vi "FIFO.WRITE.vi"(0 "FIFO In":string, 5 "FIFO Name":string, 7 "Data Type":string, 9 "Element":variant, 11 "Input Valid":bool) -> (4 "FIFO Out":string, 6 "Ready for Input":bool)   [LabVIEW 2020]
doc: "Stand-in for an FPGA FIFO Write node with the handshake interface (FIFO In, Element, Input Valid -> Ready for Input, FIFO Out) so that a VI using it can be round-tripped through AIXML. The FIFO's configuration is given as constants on the diagram: FIFO Name (the FIFO item in the LabVIEW project, e.g. TS-Filter.Command) and Data Type (the element type, e.g. orderbook.command.ctl); Element is a Variant so one VI serves every element type (wire the element through To Variant). On My Computer it only passes FIFO In to FIFO Out and reports Ready for Input = TRUE. In the FPGA VI, replace each call with the real FIFO Method Node for FIFO Name and delete the constants."
panel:
  out "Data Type (cfg)":string
  out "FIFO Name (cfg)":string
  out "Input Valid (last)":bool
  out "Element (last)":variant
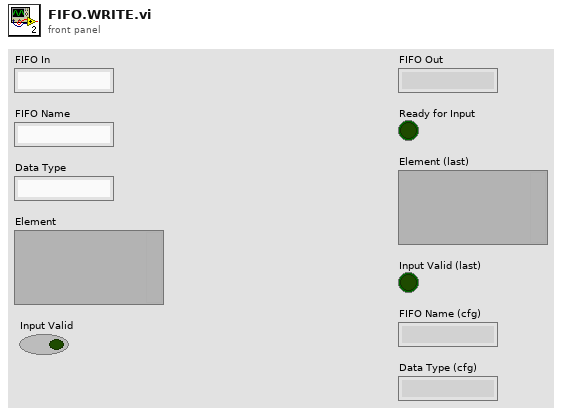
[diagram p1: front panel]
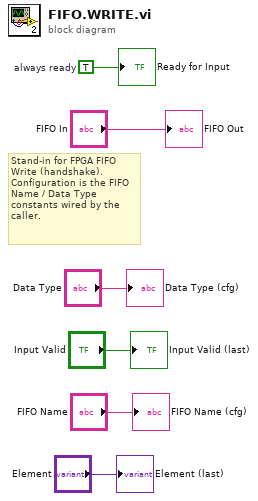
[diagram p0: block diagram]
diagram:
  w5 = TRUE  # always ready
  # "Stand-in for FPGA FIFO Write (handshake). Configuration is the FIFO Name / Data Type constants wired by the caller."
  "FIFO Out" <- "FIFO In"
  "Ready for Input" <- w5
  "Element (last)" <- "Element"
  "Input Valid (last)" <- "Input Valid"
  "FIFO Name (cfg)" <- "FIFO Name"
  "Data Type (cfg)" <- "Data Type"
